vi "Read from Data Source.vi"(7 "Project Store in":refnum<class "Project Store-INI.lvclass">, 8 "error in (no error)":errorcluster) -> (0 "error out":errorcluster, 5 "Project Store out":refnum<class "Project Store-INI.lvclass">)   [LabVIEW 2026, in "Project Store-INI.lvclass"]
doc: "Replaces the in-memory projects and tasks with the content of Projects.ini and Tasks.ini in the data folder. A file that does not exist reads as an empty table. The Project Name label in Tasks.ini is ignored - names are looked up by ID.\n\nGenerated by: Claude"
uses:
  Project Store-INI.lvclass
  Project Store-INI.lvclass/Project Store-INI.ctl
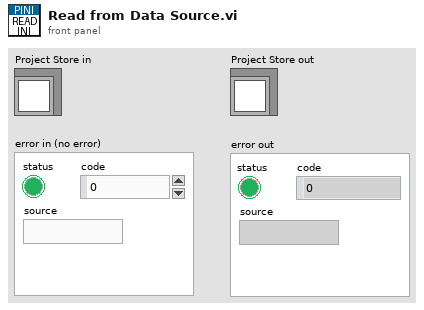
[diagram p1: front panel]
types:
  T1 = cluster{"String":string, string, string, bool, i32}
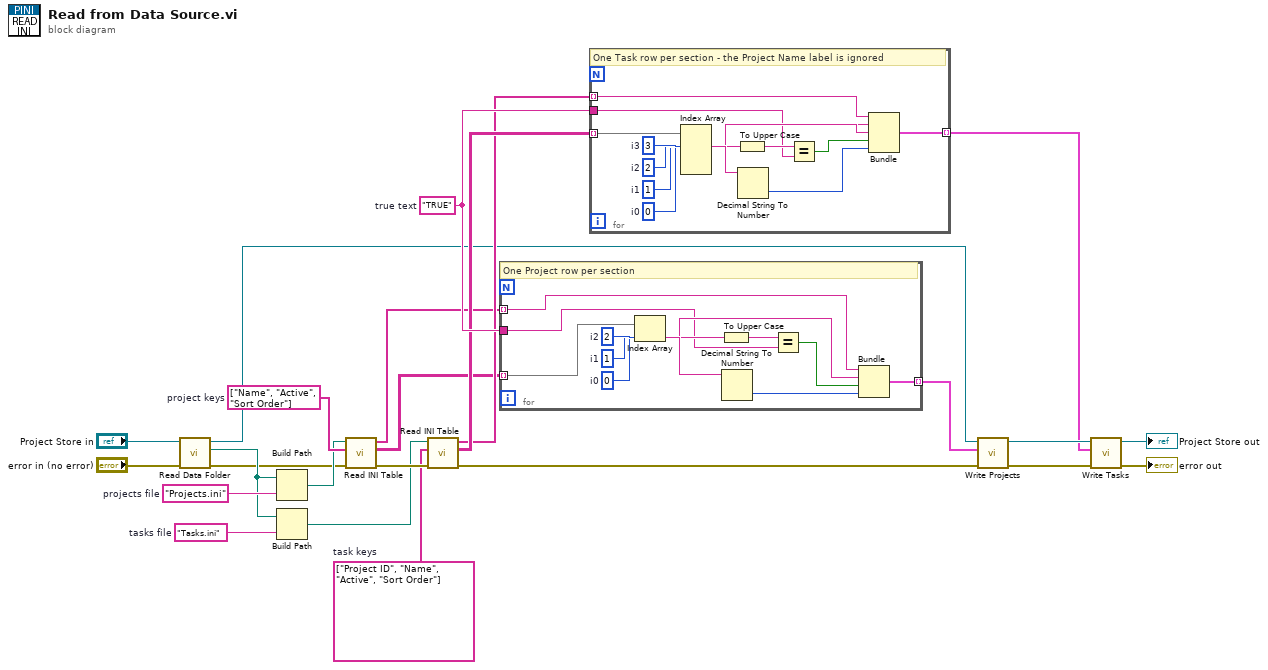
[diagram p0: block diagram]
diagram:
  w18 = "TRUE"  # true text
  w11 = string[] ["Project ID", "Name", "Active", "Sort Order"]  # task keys
  w10 = string[] ["Name", "Active", "Sort Order"]  # project keys
  w7 = "Tasks.ini"  # tasks file
  w6 = "Projects.ini"  # projects file
  n1 = call-dynamic "Read Data Folder.vi"("error in (no error)"="error in (no error)", "Project Store-INI in"="Project Store in") -> ("error out"=w3:errorcluster, "Data Folder"=w5:path, "Project Store-INI out"=w4:refnum<class "Project Store-INI.lvclass">)  [unwired: 7 in]
  n2 = Build Path(base path=w5, name or relative path=w6) -> (appended path=w8:path)
  n3 = Build Path(base path=w5, name or relative path=w7) -> (appended path=w9:path)
  n4 = call "Read INI Table.vi"("error in (no error)"=w3, "Keys"=w10, "File Path"=w8) -> ("error out"=w14:errorcluster, "Values"=w13:string[][], "Section Names"=w12:string[])  [unwired: 6 in]
  n5 = call "Read INI Table.vi"("error in (no error)"=w14, "Keys"=w11, "File Path"=w9) -> ("error out"=w17:errorcluster, "Values"=w16:string[][], "Section Names"=w15:string[])  [unwired: 6 in]
  n6 = for {
    tunnel: w18 -> [w27]
    tunnel: w12 -> [w25] mode=indexing
    tunnel: w13 -> [w26] mode=indexing
    tunnel: [w37] -> w19 mode=indexing
    w30 = 2  # i2
    w29 = 1  # i1
    w28 = 0  # i0
    # "One Project row per section"
    n7 = Index Array(array=w26, index #1=w28, index #2=w29, index #3=w30) -> (element #1=w31:string, element #2=w32:string, element #3=w33:string)
    n8 = To Upper Case(1:w32) -> (0:w34:string)
    n9 = Decimal String To Number(string=w33) -> (number=w36:i32)  [unwired: 2 in, 1 out]
    n10 = Equal?(x=w34, y=w27) -> (x = y?=w35:bool)
    n11 = Bundle("String"=w25, w31, w35, w36) -> (w37:cluster{"String":string, string, bool, i32})  [unwired: 1 in]
  }
  n12 = for {
    tunnel: w18 -> [w40]
    tunnel: w15 -> [w38] mode=indexing
    tunnel: w16 -> [w39] mode=indexing
    tunnel: [w52] -> w20 mode=indexing
    w44 = 3  # i3
    w43 = 2  # i2
    w42 = 1  # i1
    w41 = 0  # i0
    # "One Task row per section - the Project Name label is ignored"
    n13 = Index Array(array=w39, index #1=w41, index #2=w42, index #3=w43, index #4=w44) -> (element #1=w45:string, element #2=w46:string, element #3=w47:string, element #4=w48:string)  [unwired: 3 in, 3 out]
    n14 = To Upper Case(1:w47) -> (0:w49:string)
    n15 = Decimal String To Number(string=w48) -> (number=w51:i32)  [unwired: 2 in, 1 out]
    n16 = Equal?(x=w49, y=w40) -> (x = y?=w50:bool)
    n17 = Bundle("String"=w38, w45, w46, w50, w51) -> (w52:T1)  [unwired: 1 in]
  }
  n18 = call-dynamic "Write Projects.vi"("error in (no error)"=w17, "Project List"=w19, "Project Store in"=w4) -> ("error out"=w21:errorcluster, "Project Store out"=w22:refnum<class "Project Store-INI.lvclass">)  [unwired: 7 in]
  n19 = call-dynamic "Write Tasks.vi"("error in (no error)"=w21, "Task List"=w20, "Project Store in"=w22) -> ("error out"=→"error out":errorcluster, "Project Store out"=→"Project Store out":refnum<class "Project Store-INI.lvclass">)  [unwired: 7 in]
